vi "AssertVIExecState_Tests.vi"(11 "error in":errorcluster) -> (15 "error out":errorcluster)   [LabVIEW 2016, in "DronaTest.lvlib"]
uses:
  DronaTest.lvlib
  APIs/Assert/AssertVI/Exec/AssertVIExecNotBad.vi
  <vilib>/addons/_JKI Toolkits/Caraya/classes/Assert/Assert True.vi
  APIs/Assert/AssertVI/Exec/AssertVIExecRunning.vi
  APIs/Stimulus/VI/CloseVI.vi
  APIs/Assert/AssertVI/Exec/AssertVIExecIdle.vi
  <vilib>/addons/_JKI Toolkits/Caraya/classes/Test/Test.lvclass
  Drona.lvlib
  <vilib>/addons/_JKI Toolkits/Caraya/classes/Assert/Assert.lvclass
  APIs/Stimulus/VI/VI.lvlib
  APIs/Assert/AssertVI/AssertVI.lvlib
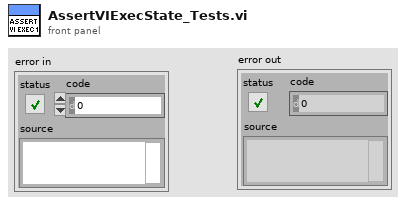
[diagram p1: front panel]
types:
  T1 = enum32{"Bad", "Idle", "Run top level", "Running"}
  T2 = enum32{"Bad", "Idle", "Run top level", "Running"}[]
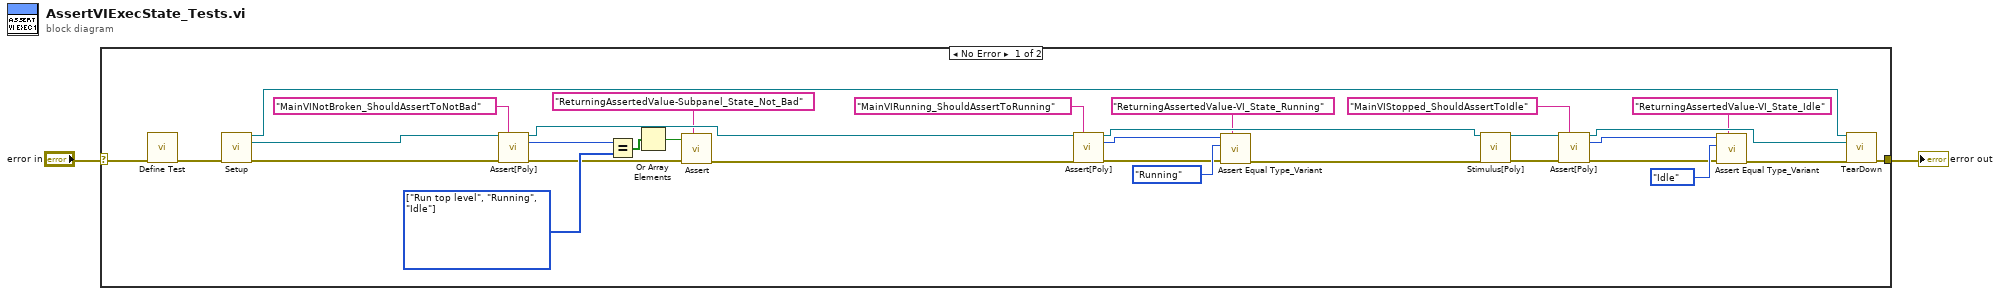
[diagram p0: block diagram]
diagram:
  n1 = case shown="No Error" "error in" {
    selector: "error in" -> [w33 w34]
    tunnel: [w20 w34] -> w1
    frame No Error {
      w9 = T2 [enum."Run top level", enum."Running", enum."Idle"] items=["Bad", "Idle", "Run top level", "Running"] ("Execution:State")
      n2 = call <vilib>:"Define Test.vi"("error in (no error)"=w33) -> ("error out"=w30:errorcluster)  [unwired: 9 in, 1 out]
      n3 = call "Setup.vi"("error in (no error)"=w30) -> ("Application Ref"=w21:refnum<vi>, "VI out"=w24:refnum<vi>, "error out"=w25:errorcluster)  [unwired: 12 in]
      n4 = call-poly "Assert[Poly].vi"("VI Reference In"=w24, "Test Label"="MainVINotBroken_ShouldAssertToNotBad" ("Label"), "Error In"=w25) -> ("VI Reference Out"=w23:refnum<vi>, "Asserted Value"=w7:T1, "Error Out"=w6:errorcluster)  [unwired: 10 in]
      n5 = Equal?(x=w7, y=w9) -> (x = y?=w10:bool[])
      n6 = Or Array Elements(Boolean array=w10) -> (logical OR=w11:bool)
      n7 = call-poly <vilib>:"Assert.vi"("Label"="ReturningAssertedValue-Subpanel_State_Not_Bad", "error in (no error)"=w6, "True?"=w11) -> ("error out"=w3:errorcluster)  [unwired: 7 in, 1 out]
      n8 = call-poly "Assert[Poly].vi"("VI Reference In"=w23, "Test Label"="MainVIRunning_ShouldAssertToRunning" ("Label"), "Error In"=w3) -> ("VI Reference Out"=w22:refnum<vi>, "Asserted Value"=w13:T1, "Error Out"=w15:errorcluster)  [unwired: 10 in]
      n9 = call <vilib>:"Assert Equal Type_Variant.vi"("Label"="ReturningAssertedValue-VI_State_Running", "error in (no error)"=w15, "Y"=T1."Running" ("Asserted Value"), "X"=w13) -> ("error out"=w14:errorcluster)  [unwired: 6 in, 1 out]
      n10 = call-poly "Stimulus[Poly].vi"("VI Reference In"=w22, "error in"=w14) -> ("VI Reference Out"=w28:refnum<vi>, "error out"=w29:errorcluster)  [unwired: 12 in]
      n11 = call-poly "Assert[Poly].vi"("VI Reference In"=w28, "Test Label"="MainVIStopped_ShouldAssertToIdle" ("Label"), "Error In"=w29) -> ("VI Reference Out"=w26:refnum<vi>, "Asserted Value"=w17:T1, "Error Out"=w5:errorcluster)  [unwired: 10 in]
      n12 = call <vilib>:"Assert Equal Type_Variant.vi"("Label"="ReturningAssertedValue-VI_State_Idle", "error in (no error)"=w5, "Y"=T1."Idle" ("Asserted Value"), "X"=w17) -> ("error out"=w4:errorcluster)  [unwired: 6 in, 1 out]
      n13 = call "TearDown.vi"("Application Ref"=w21, "VI in"=w26, "error in (no error)"=w4) -> ("error out"=w20:errorcluster)  [unwired: 12 in]
    }
    frame Error {
    }
  }
  "error out" <- w1
